vi "Call_UseXctAnalysisDLL.vi"   [LabVIEW 2015]
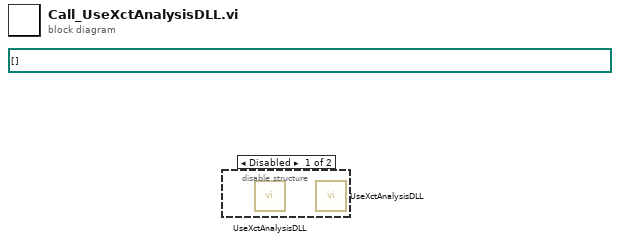
[diagram p0: block diagram]
diagram:
  (unwired) path[] []
  n1 = disable-structure shown="Disabled" {
    frame Disabled {
      n2 = call "UseXctAnalysisDLL.vi"() -> ()  [unwired: 12 in]
      n3 = call "UseXctAnalysisDLL.vi"() -> ()  [unwired: 12 in]
    }
    frame Enabled {
    }
  }
